vi "RemoteVI New Token.vi"(11 "error in":errorcluster) -> (4 "token":string, 15 "error out":errorcluster)   [LabVIEW 2020, in "RemoteVI.lvlib"]
doc: "Makes a new access token for a share (docs\\security.md): 16 bytes from the operating system's cryptographically secure random number generator (bcrypt BCryptGenRandom.vi), written as 32 lowercase hex digits. error out carries error in and the error of the call; an NTSTATUS other than 0 is error 5003 and token is empty, so a share never starts with a guessable token."
uses:
  RemoteVI.lvlib
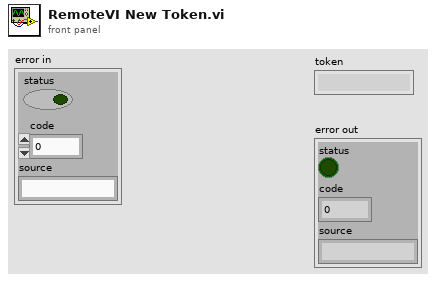
[diagram p1: front panel]
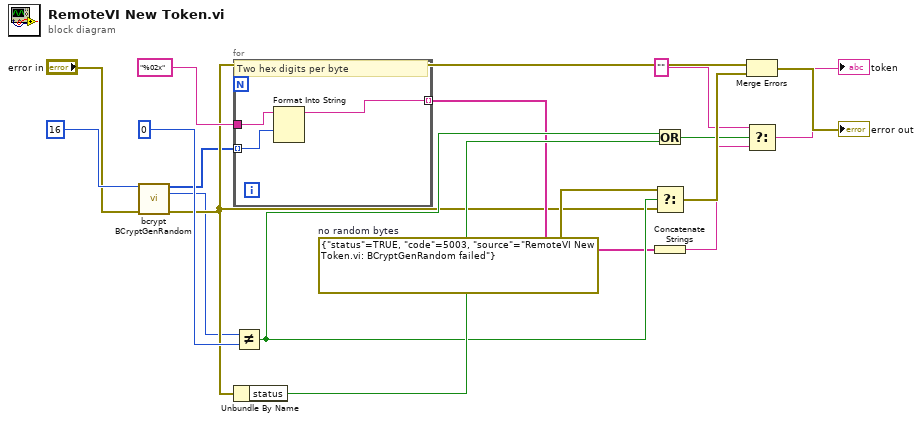
[diagram p0: block diagram]
diagram:
  w15 = errorcluster {"status"=TRUE, "code"=5003, "source"="RemoteVI New Token.vi: BCryptGenRandom failed"}  # no random bytes
  n1 = call "bcrypt BCryptGenRandom.vi"("byte count"=u32 16, "error in"="error in") -> ("random bytes"=w3:u8[], "return value"=w4:i32, "error out"=w5:errorcluster)  [unwired: 11 in]
  n2 = for {
    tunnel: "%02x" -> [w19]
    tunnel: w3 -> [w18] mode=indexing
    tunnel: [w20] -> w7 mode=indexing
    # "Two hex digits per byte"
    n3 = Format Into String(format string=w19, w18) -> (resulting string=w20:string)  [unwired: 2 in, 1 out]
  }
  n4 = Not Equal?(x=w4, y=0) -> (x != y?=w10:bool)
  n5 = Unbundle By Name(w5) -> ("status"=w11:bool)
  n6 = Or(x=w10, y=w11) -> (x .or. y?=w12:bool)
  n7 = Select(t=w15, s=w10, f=w5) -> (s? t:f=w16:errorcluster)
  n8 = Concatenate Strings(w7) -> (w8:string)
  n9 = Merge Errors(w5, w16) -> (→"error out":errorcluster)
  n10 = Select(t="", s=w12, f=w8) -> (s? t:f=→"token":string)
